vi "Read current vs temperature_3ch_2.1___.vi"(8 "stop":bool) -> (1 "X1":cluster{"Y":dbl[], "Y":dbl[]}[](graph), 3 "Temp vs Time":cluster{"Y":dbl[], "Y":dbl[]}[](graph), 5 "X4":cluster{"Y":dbl[], "Y":dbl[]}[](graph))   [LabVIEW 2013]
uses:
  <userlib>/LevyLab/DAQ-Lockin-SubVI/Lock-in Globles.vi
  P:/users1/Joe/Lockin-4461_3.0 4461-4462 Multichannel Folder/DAQ-Lockin-SubVI/Lock-in Globles Multiple Inputs and Outputs.vi
  <userlib>/LevyLab/PPMS VI/SubVI/ITX_Global.vi
  Q:/inst/Leiden measurements VIs/IV measurement/Sub VIs/Global Value.vi
panel:
  in  "Tab Control":T1(tab)
  in  "milliseconds to wait":u32=1000
  in  "Comments":string="SA02610M 20130128\ncool down\n"
  out "Connected":string="I-:4\nV2+:28\nI+:1\nV1+:2\nV-:3\nV2-:5\n"
  in  "Lockins":i32[](array[numeric])
  out "OSC Configuration 2":T2(array[cluster])=[[{"Signal Type"=enum."Sine Wave", "DC"=0.0003, "Amplitude"=0.0005, "frequency"=1.3459999999999999, "Phase"=0.0}, {"Signal Type"=enum."Sine Wave", "DC"=0.0, "Amplitude"=0.0, "frequency"=1.346, "Phase"=0.0}, {"Signal Type"=enum."Sine Wave", "DC"=0.0, "Amplitude"=0.0, "frequency"=1.346, "Phase"=0.0}, {"Signal Type"=enum."Sine Wave", "DC"=0.0, "Amplitude"=0.0, "frequency"=1.346, "Phase"=0.0}]] {"frequency" step=0.001 format="%.3p"; "Amplitude" format="%0.2p"; "DC" min=-0.99 max=0.99 format="%.2p"}
  out "Y 0":cluster{"Y":dbl[], "Y":dbl[]}[](graph)
  out "X 0":cluster{"Y":dbl[], "Y":dbl[]}[](graph)
  out "Y1":cluster{"Y":dbl[], "Y":dbl[]}[](graph)
  out "X2":cluster{"Y":dbl[], "Y":dbl[]}[](graph)
  out "Y2":cluster{"Y":dbl[], "Y":dbl[]}[](graph)
  out "X3":cluster{"Y":dbl[], "Y":dbl[]}[](graph)
  out "Y3":cluster{"Y":dbl[], "Y":dbl[]}[](graph)
  out "Y4":cluster{"Y":dbl[], "Y":dbl[]}[](graph)
  out "X5":cluster{"Y":dbl[], "Y":dbl[]}[](graph)
  out "Y5":cluster{"Y":dbl[], "Y":dbl[]}[](graph)
  out "R":cluster{"Y":dbl[], "Y":dbl[]}[](graph)
  in  "V1":i32
  in  "Current":i32
  in  "V2":i32
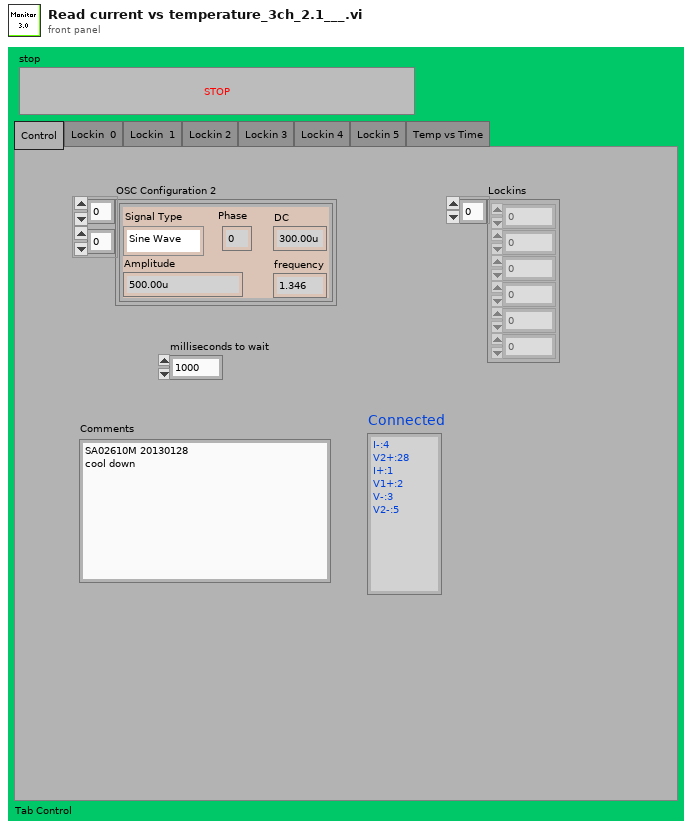
[diagram p1: front panel]
types:
  T1 = enum32{"Control", "Lockin  0", "Lockin  1", "Lockin 2", "Lockin 3", "Lockin 4", "Lockin 5", "Temp vs Time"}
  T2 = cluster{"Signal Type":enum16{"Sine Wave", "Triangle Wave", "Square Wave", "Sawtooth Wave"}, "DC":dbl, "Amplitude":dbl, "frequency":dbl, "Phase":dbl}[][]
  T3 = cluster{"Signal Type":enum16{"Sine Wave", "Triangle Wave", "Square Wave", "Sawtooth Wave"}, "DC":dbl, "Amplitude":dbl, "frequency":dbl, "Phase":dbl}[]
  T4 = cluster{"Signal Type":enum16{"Sine Wave", "Triangle Wave", "Square Wave", "Sawtooth Wave"}, "DC":dbl, "Amplitude":dbl, "frequency":dbl, "Phase":dbl}
  T5 = cluster{"Channel":u16, "Gain":u16, "Shunt Resistor":u16, "Measure":u16}[]
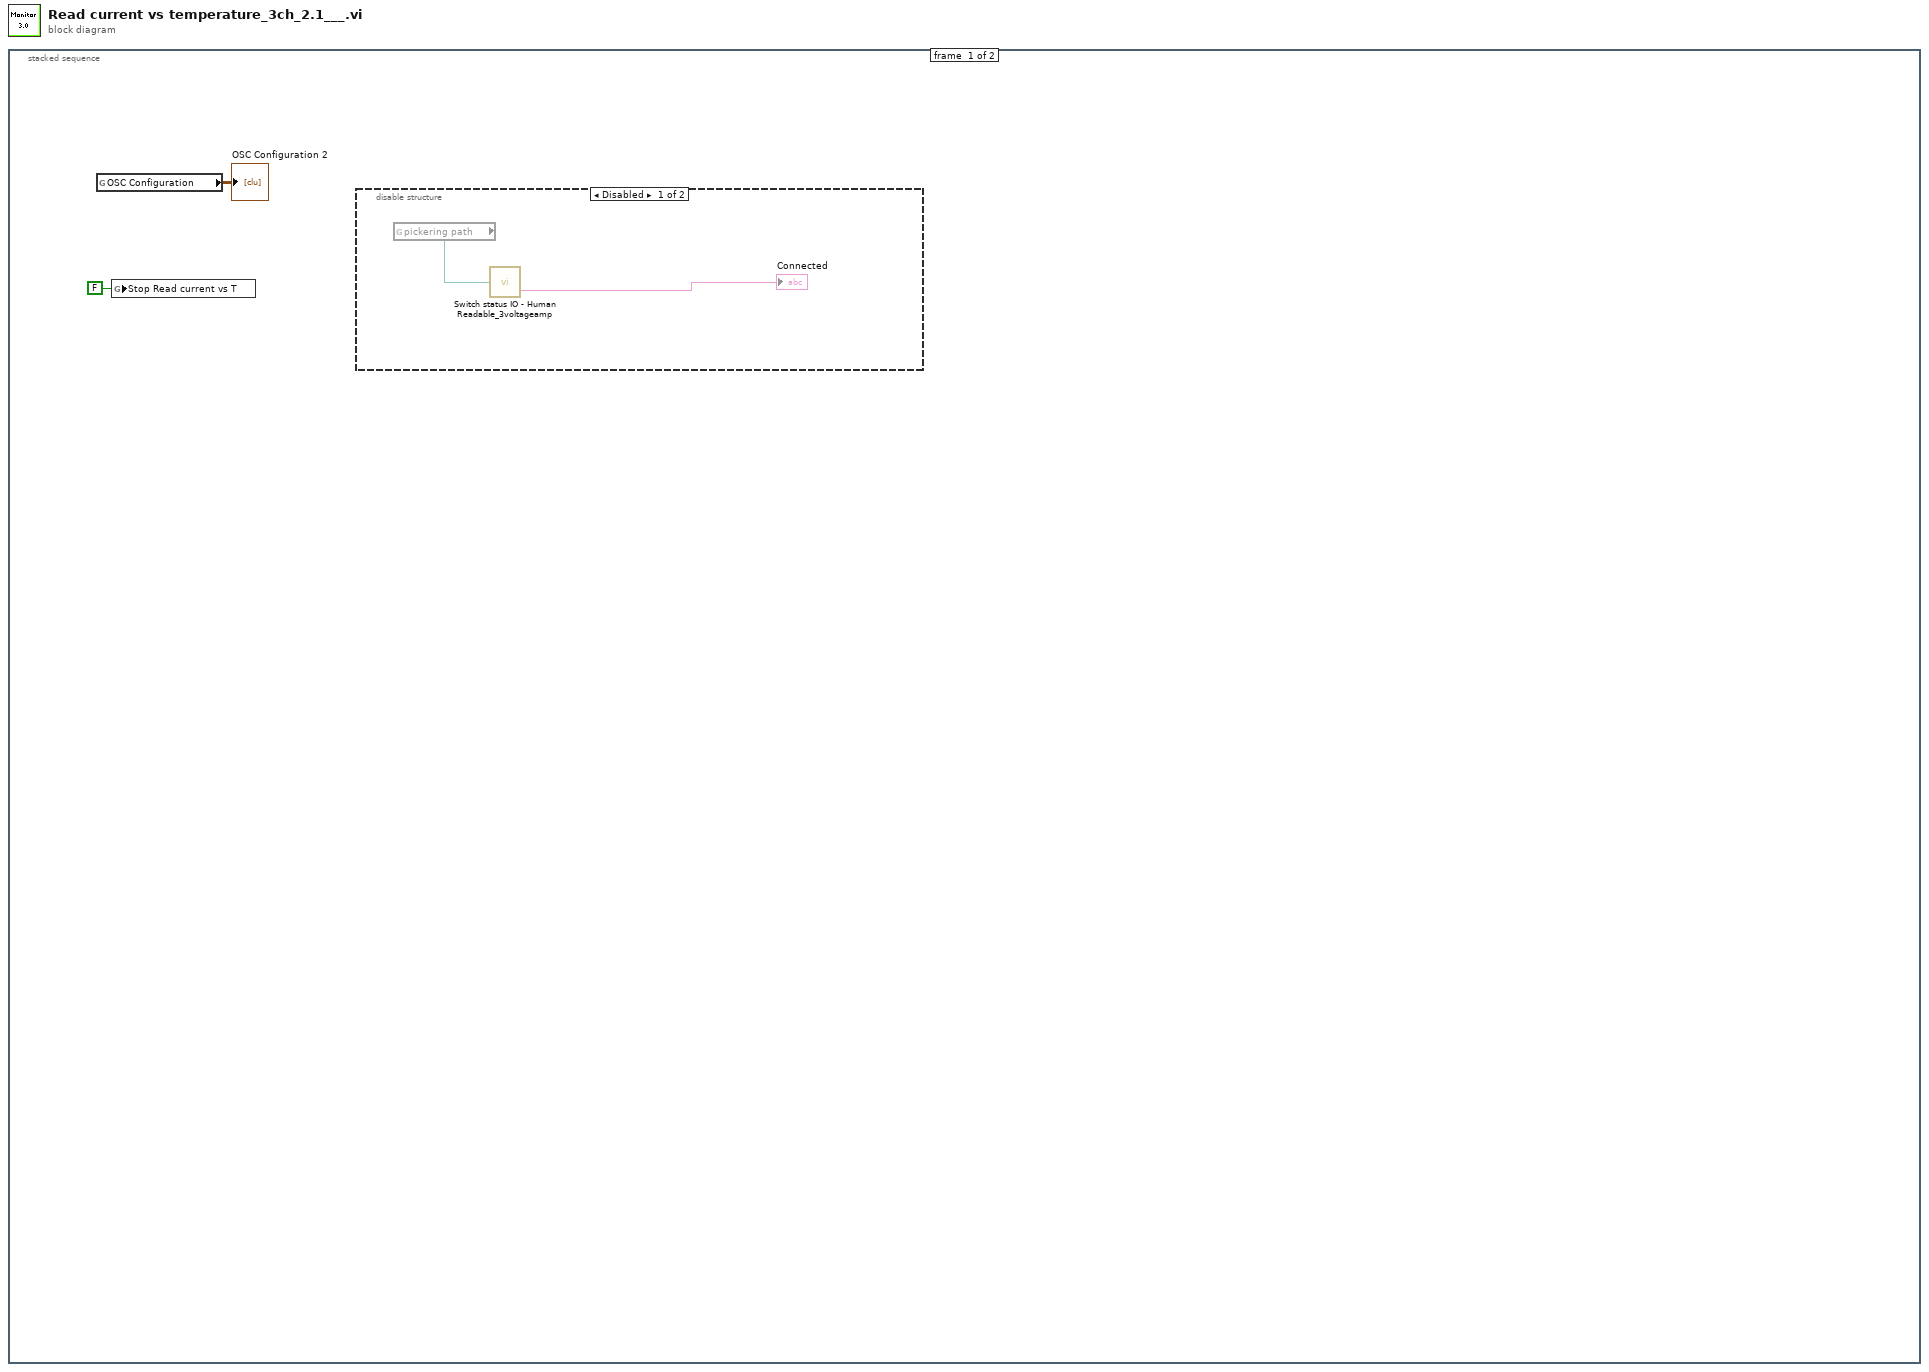
[diagram p0: block diagram]
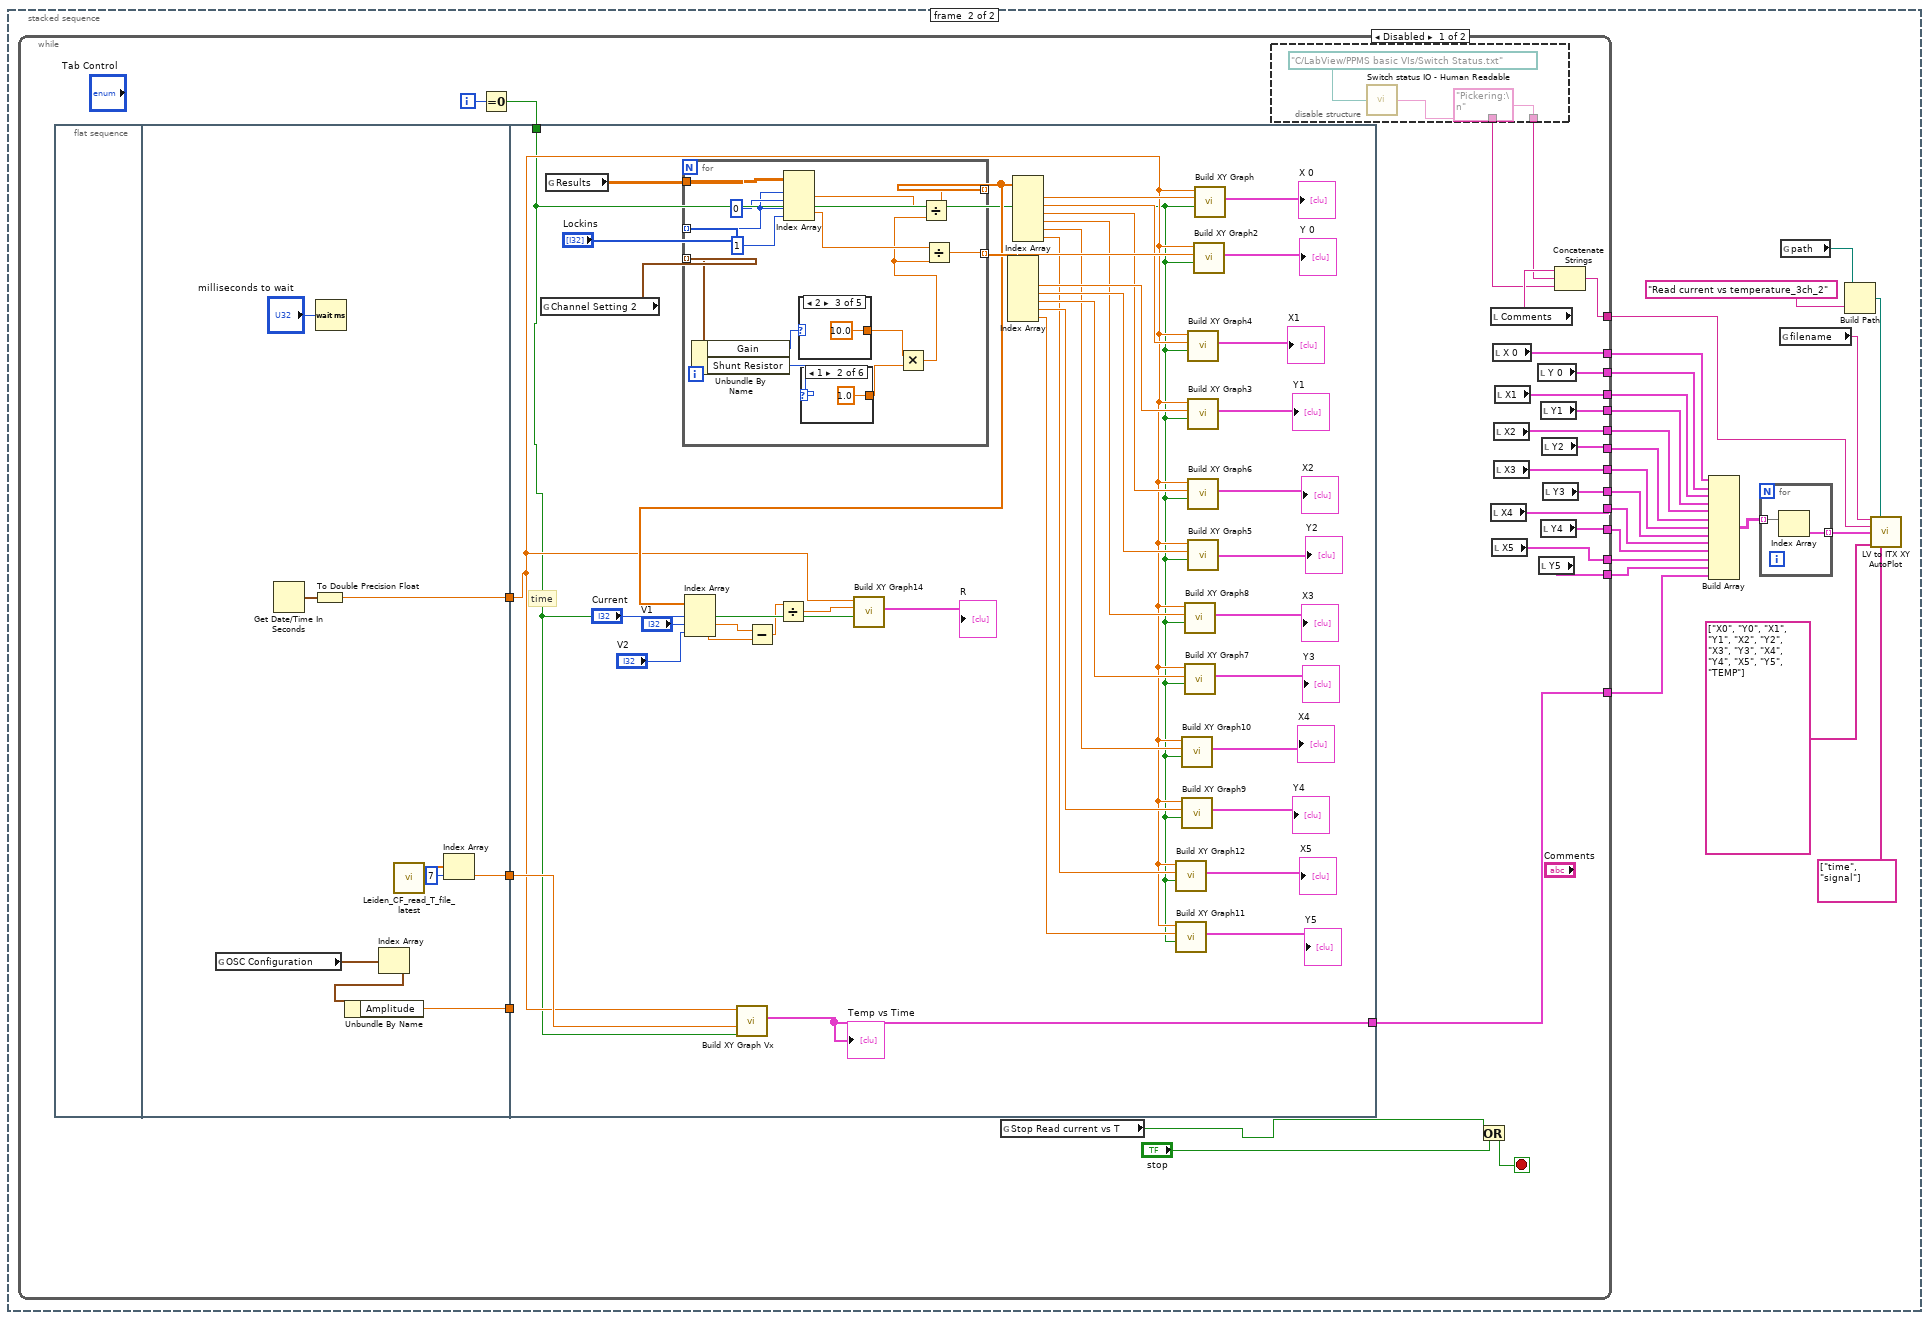
[diagram p3: hidden frame]
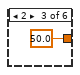
[diagram p6: hidden frame]
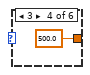
[diagram p7: hidden frame]
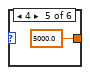
[diagram p8: hidden frame]
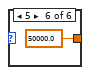
[diagram p9: hidden frame]
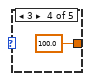
[diagram p12: hidden frame]
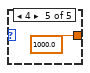
[diagram p13: hidden frame]
diagram:
  n1 = stacked-sequence {
    frame #0 {
      n2 = global read "Lock-in Globles Multiple Inputs and Outputs.vi" "OSC Configuration"() -> (→"OSC Configuration 2":T2)
      n3 = global write "Lock-in Globles.vi" "Stop Read current vs T"(FALSE ("Stop Read current vs T")) -> ()
      n4 = disable-structure shown="Disabled" {
        frame Disabled {
          n5 = global read "ITX_Global.vi" "pickering path"() -> (w3:path)
          n6 = call <userlib>:"Switch status IO - Human Readable_3voltageamp.vi"("Switch status"=w3) -> ("String"=→"Connected":string)  [unwired: 3 in]
        }
        frame Enabled {
        }
      }
    }
    frame #1 {
      n7 = while {
        tunnel: [w48] -> w26
        tunnel: [w47] -> w25
        tunnel: [w37] -> w24
        tunnel: [w35] -> w13
        tunnel: [w46] -> w20
        tunnel: [w36] -> w14
        tunnel: [w32] -> w12
        tunnel: [w31] -> w11
        tunnel: [w30] -> w10
        tunnel: [w29] -> w9
        tunnel: [w39] -> w8
        tunnel: [w38] -> w7
        tunnel: [w34] -> w6
        tunnel: [w33] -> w5
        i -> [w53]
        stop <- w50 stop-if-true
        n8 = flat-sequence {
          tunnel: [w63] -> w51
          tunnel: [w60] -> w41
          tunnel: [w57] -> w40
          tunnel: w52 -> [w69]
          tunnel: w51 -> [w73]
          tunnel: w41 -> [_]
          tunnel: w40 -> [w107]
          tunnel: [w106] -> w39
          frame #0 {
          }
          frame #1 {
            n9 = global read "Lock-in Globles.vi" "OSC Configuration"() -> (w62:T3)
            n10 = Get Date/Time In Seconds() -> (seconds since 1Jan1904=w64:timestamp)
            n11 = To Double Precision Float(number=w64) -> (double precision float=w63:dbl)
            n12 = Wait (ms)(milliseconds to wait="milliseconds to wait") -> ()  [unwired: 1 out]
            n13 = Index Array(array=w62) -> (element=w61:T4)  [unwired: 1 in]
            n14 = Unbundle By Name(w61) -> ("Amplitude"=w60:dbl)
            n15 = call "Leiden_CF_read_T_file_latest.vi"() -> ("T array"=w59:dbl[])  [unwired: 11 in]
            n16 = Index Array(array=w59, index=7) -> (element=w57:dbl)
          }
          frame #2 {
            # "time"
            n17 = global read "Global Value.vi" "Channel Setting 2"() -> (w78:T5)
            n18 = global read "Lock-in Globles Multiple Inputs and Outputs.vi" "Results"() -> (w105:dbl[][])
            n19 = for {
              tunnel: w105 -> [w118]
              tunnel: "Lockins" -> [w119] mode=indexing
              tunnel: [w111] -> w77 mode=indexing
              tunnel: [w108] -> w103 mode=indexing
              tunnel: w78 -> [w116] mode=indexing
              n20 = Unbundle By Name(w116) -> ("Gain"=w117:u16, "Shunt Resistor"=w115:u16)
              n21 = Index Array(array=w118, index (row) #1=w119, index (col) #1=0 ("disabled index (col)"), index (row) #2=w119, index (col) #2=1 ("disabled index (col)")) -> (element #1=w112:dbl, element #2=w110:dbl)
              n22 = case shown="2" w117 {
                selector: w117 -> [w128 w129 _ _ _]
                tunnel: [w128 w129 10.0 100.0 1000.0] -> w114
                frame 0, Default {
                }
                frame 1 {
                }
                frame 2 {
                }
                frame 3 {
                }
                frame 4 {
                }
              }
              n23 = case shown="1" w115 {
                selector: w115 -> [w122 _ _ _ _ _]
                tunnel: [w122 1.0 50.0 500.0 5000.0 50000.0] -> w113
                frame 0, Default {
                }
                frame 1 {
                }
                frame 2 {
                }
                frame 3 {
                }
                frame 4 {
                }
                frame 5 {
                }
              }
              n24 = Multiply(x=w114, y=w113) -> (x*y=w109:dbl)
              n25 = Divide(x=w112, y=w109) -> (x/y=w111:dbl)
              n26 = Divide(x=w110, y=w109) -> (x/y=w108:dbl)
            }
            n27 = Index Array(array=w77, index #1="Current", index #2="V1", index #3="V2") -> (element #1=w66:dbl, element #2=w72:dbl, element #3=w71:dbl)
            n28 = call "Build XY Graph Vx"("Reset"=w69, "Y Input"=w107, "X Input"=w73) -> ("XY Graph"=w106:cluster{"Y":dbl[], "Y":dbl[]}[])  [unwired: 2 in, 6 out]
            "Temp vs Time" <- w106
            n29 = Subtract(x=w72, y=w71) -> (x-y=w67:dbl)
            n30 = Divide(x=w67, y=w66) -> (x/y=w70:dbl)
            n31 = call "Build XY Graph14"("Reset"=w69, "Y Input"=w70, "X Input"=w73) -> ("XY Graph"=→"R":cluster{"Y":dbl[], "Y":dbl[]}[])  [unwired: 2 in, 6 out]
            n32 = Index Array(array=w103) -> (element #1=w101:dbl, element #2=w97:dbl, element #3=w93:dbl, element #4=w89:dbl, element #5=w85:dbl, element #6=w81:dbl)  [unwired: 6 in]
            n33 = Index Array(array=w77) -> (element #1=w102:dbl, element #2=w98:dbl, element #3=w94:dbl, element #4=w90:dbl, element #5=w86:dbl, element #6=w82:dbl)  [unwired: 6 in]
            n34 = call "Build XY Graph12"("Reset"=w69, "Y Input"=w82, "X Input"=w73) -> ("XY Graph"=→"X5":cluster{"Y":dbl[], "Y":dbl[]}[])  [unwired: 2 in, 6 out]
            n35 = call "Build XY Graph11"("Reset"=w69, "Y Input"=w81, "X Input"=w73) -> ("XY Graph"=→"Y5":cluster{"Y":dbl[], "Y":dbl[]}[])  [unwired: 2 in, 6 out]
            n36 = call "Build XY Graph10"("Reset"=w69, "Y Input"=w86, "X Input"=w73) -> ("XY Graph"=→"X4":cluster{"Y":dbl[], "Y":dbl[]}[])  [unwired: 2 in, 6 out]
            n37 = call "Build XY Graph9"("Reset"=w69, "Y Input"=w85, "X Input"=w73) -> ("XY Graph"=→"Y4":cluster{"Y":dbl[], "Y":dbl[]}[])  [unwired: 2 in, 6 out]
            n38 = call "Build XY Graph8"("Reset"=w69, "Y Input"=w90, "X Input"=w73) -> ("XY Graph"=→"X3":cluster{"Y":dbl[], "Y":dbl[]}[])  [unwired: 2 in, 6 out]
            n39 = call "Build XY Graph7"("Reset"=w69, "Y Input"=w89, "X Input"=w73) -> ("XY Graph"=→"Y3":cluster{"Y":dbl[], "Y":dbl[]}[])  [unwired: 2 in, 6 out]
            n40 = call "Build XY Graph4"("Reset"=w69, "Y Input"=w98, "X Input"=w73) -> ("XY Graph"=→"X1":cluster{"Y":dbl[], "Y":dbl[]}[])  [unwired: 2 in, 6 out]
            n41 = call "Build XY Graph3"("Reset"=w69, "Y Input"=w97, "X Input"=w73) -> ("XY Graph"=→"Y1":cluster{"Y":dbl[], "Y":dbl[]}[])  [unwired: 2 in, 6 out]
            n42 = call "Build XY Graph6"("Reset"=w69, "Y Input"=w94, "X Input"=w73) -> ("XY Graph"=→"X2":cluster{"Y":dbl[], "Y":dbl[]}[])  [unwired: 2 in, 6 out]
            n43 = call "Build XY Graph5"("Reset"=w69, "Y Input"=w93, "X Input"=w73) -> ("XY Graph"=→"Y2":cluster{"Y":dbl[], "Y":dbl[]}[])  [unwired: 2 in, 6 out]
            n44 = call "Build XY Graph2"("Reset"=w69, "Y Input"=w101, "X Input"=w73) -> ("XY Graph"=→"Y 0":cluster{"Y":dbl[], "Y":dbl[]}[])  [unwired: 2 in, 6 out]
            n45 = call "Build XY Graph"("Reset"=w69, "Y Input"=w102, "X Input"=w73) -> ("XY Graph"=→"X 0":cluster{"Y":dbl[], "Y":dbl[]}[])  [unwired: 2 in, 6 out]
          }
        }
        n46 = Equal To 0?(x=w53) -> (x = 0?=w52:bool)
        n47 = global read "Lock-in Globles.vi" "Stop Read current vs T"() -> (w42:bool)
        n48 = disable-structure shown="Disabled" {
          disable-tunnel: ["Pickering:\n" ("string") _] -> w44
          disable-tunnel: [w54 _] -> w43
          frame Disabled {
            n49 = call <userlib>:"Switch status IO - Human Readable.vi"("Switch status"=path "C:/LabView/PPMS basic VIs/Switch Status.txt") -> ("String"=w54:string)
          }
          frame Enabled {
          }
        }
        n50 = Or(x=w42, y="stop") -> (x .or. y?=w50:bool)
        n51 = local read "Comments"() -> (w45:string)
        n52 = local read "X4"() -> (w32:cluster{"Y":dbl[], "Y":dbl[]}[])
        n53 = local read "X5"() -> (w30:cluster{"Y":dbl[], "Y":dbl[]}[])
        n54 = local read "X 0"() -> (w48:cluster{"Y":dbl[], "Y":dbl[]}[])
        n55 = local read "X2"() -> (w36:cluster{"Y":dbl[], "Y":dbl[]}[])
        n56 = local read "X3"() -> (w34:cluster{"Y":dbl[], "Y":dbl[]}[])
        n57 = local read "X1"() -> (w38:cluster{"Y":dbl[], "Y":dbl[]}[])
        n58 = local read "Y 0"() -> (w47:cluster{"Y":dbl[], "Y":dbl[]}[])
        n59 = local read "Y5"() -> (w29:cluster{"Y":dbl[], "Y":dbl[]}[])
        n60 = local read "Y1"() -> (w37:cluster{"Y":dbl[], "Y":dbl[]}[])
        n61 = local read "Y4"() -> (w31:cluster{"Y":dbl[], "Y":dbl[]}[])
        n62 = local read "Y2"() -> (w35:cluster{"Y":dbl[], "Y":dbl[]}[])
        n63 = local read "Y3"() -> (w33:cluster{"Y":dbl[], "Y":dbl[]}[])
        n64 = Concatenate Strings(w45, w44, w43) -> (w46:string)
      }
      n65 = Build Array(w26, w25, w7, w24, w14, w13, w6, w5, w12, w11, w10, w9, w8) -> (w23:cluster{"Y":dbl[], "Y":dbl[]}[][])
      n66 = for {
        tunnel: w23 -> [w28] mode=indexing
        tunnel: [w27] -> w22 mode=indexing
        n67 = Index Array(array=w28) -> (element=w27:cluster{"Y":dbl[], "Y":dbl[]})  [unwired: 1 in]
      }
      n68 = global read "ITX_Global.vi" "filename"() -> (w21:string)
      n69 = global read "ITX_Global.vi" "path"() -> (w17:path)
      n70 = Build Path(base path=w17, name or relative path="Read current vs temperature_3ch_2") -> (appended path=w16:path)
      n71 = call <userlib>:"LV to ITX XY AutoPlot.vi"("filename"=w21, "path"=w16, "Notes"=w20, "XY Array"=w22, "wavenames (.Vx, etc)"=string[] ["X0", "Y0", "X1", "Y1", "X2", "Y2", "X3", "Y3", "X4", "Y4", "X5", "Y5", "TEMP"], "X,Y Labels"=string[] ["time", "signal"]) -> ()  [unwired: 9 in, 1 out]
    }
  }
